vi "(RAG) Retrieve Contexts from KB.vi"(0 "Python Session Refnum in":refnum<k35>, 1 "Chroma Database Folder":path, 5 "Knowledge Base Name":string, 7 "RAG Query":string, 9 "K":u32=5, 11 "error in":errorcluster, 12 "Embedding Model URL":string, 13 "Embedding Model Name":string) -> (4 "Python Session Refnum out":refnum<k35>, 6 "Retrieved Contexts":string, 15 "error out":errorcluster)   [LabVIEW 2023, in "LabVIEW RAG.lvlib"]
uses:
  LabVIEW RAG.lvlib
  AI RAG Globals.vi
  labview-ai-share/LabVIEW AI Base.lvlib
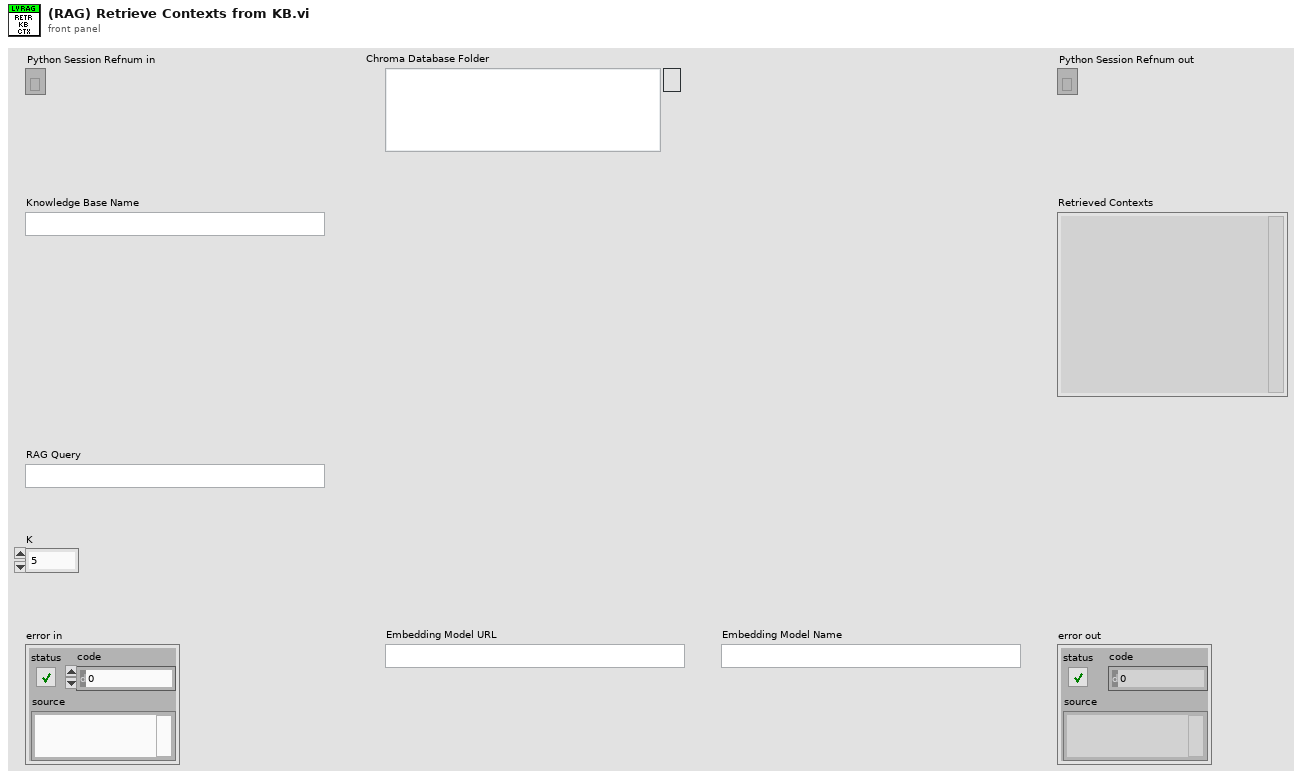
[diagram p1: front panel]
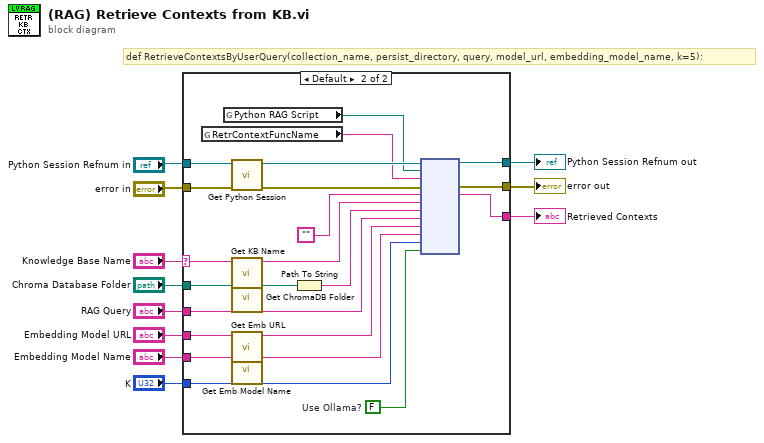
[diagram p0: block diagram]
diagram:
  # "def RetrieveContextsByUserQuery(collection_name, persist_directory, query, model_url, embedding_model_name, k=5):"
  n1 = case shown="Default" "Knowledge Base Name" {
    selector: "Knowledge Base Name" -> [_ w29]
    tunnel: "Chroma Database Folder" -> [_ w34]
    tunnel: [w13 w33] -> w10
    tunnel: [w12 w32] -> w9
    tunnel: "error in" -> [w12 w31]
    tunnel: "Python Session Refnum in" -> [w13 w30]
    tunnel: "RAG Query" -> [_ w27]
    tunnel: "Embedding Model URL" -> [_ w26]
    tunnel: "Embedding Model Name" -> [_ w25]
    tunnel: "K" -> [_ w24]
    tunnel: [_ w22] -> w1
    frame "" {
    }
    frame Default {
      w21 = FALSE  # Use Ollama?
      n2 = global read "AI RAG Globals.vi" "RetrContextFuncName"() -> (w18:string)
      n3 = global read "AI RAG Globals.vi" "Python RAG Script"() -> (w19:path)
      n4 = call "Get Python Session.vi"("Python Session in"=w30) -> ("Python Session out"=w20:refnum<k35>)  [unwired: 10 in]
      n5 = call "Get KB Name.vi"("KB Name"=w29) -> ("KB Name"=w17:string)  [unwired: 10 in]
      n6 = call "Get ChromaDB Folder.vi"("ChromaDB Folder in"=w34) -> ("ChromaDB Folder out"=w16:path)  [unwired: 10 in]
      n7 = call "Get Emb URL.vi"("Embedding Model URL in"=w26) -> ("Embedding Model URL out"=w15:string)  [unwired: 10 in]
      n8 = call "Get Emb Model Name.vi"("Embedding Model Name in"=w25) -> ("Embedding Model Name out"=w14:string)  [unwired: 10 in]
      n9 = Path To String(path=w16) -> (string=w28:string)
      n10 = node(w20, w19, w18, w31, "", w17, w28, w27, w15, w14, w24, w21) -> (w33:refnum<k35>, w32:errorcluster, w22:string)  [unwired: 7 in, 2 out]
    }
  }
  "Python Session Refnum out" <- w10
  "error out" <- w9
  "Retrieved Contexts" <- w1
